vi "t162_ten_class_links.vi"() -> ()   [LabVIEW 2019]
doc: "Two classes, eight distinct methods and one vi.lib call: the method links carry contents 9 and 10 - a TAB and a line feed. Written as literal character references they stayed six characters long in the file, and LabVIEW refused the VI with Error 74 until 2026-10-12."
uses:
  Projects/LabVIEWMCP/experiments/aixml-without-grpc/tests/fixtures/Gauge/Gauge.lvclass
  Projects/LabVIEWMCP/experiments/aixml-without-grpc/tests/fixtures/Box/Box.lvclass
panel:
  out "trimmed":string
  out "width out":dbl
  out "offset out":dbl
  out "gain out":dbl
  out "name out":string
  in  "text":string
  in  "width":dbl
  in  "offset":dbl
  in  "gain":dbl
  in  "name":string
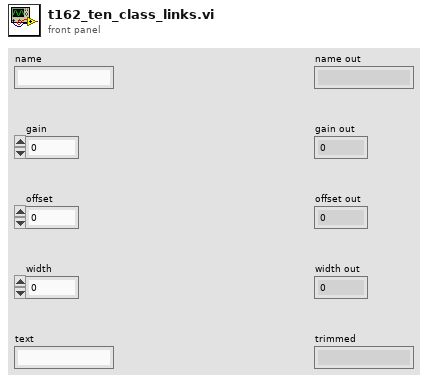
[diagram p1: front panel]
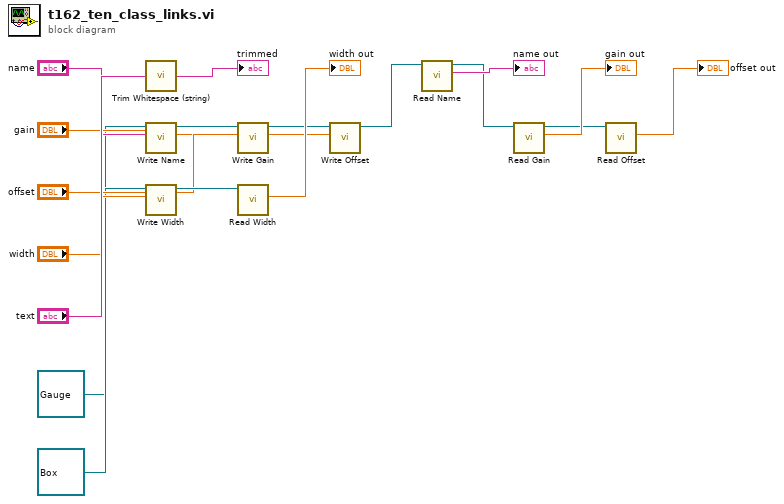
[diagram p0: block diagram]
diagram:
  n1 = call <vilib>:"Trim Whitespace (string).vi"("string"="text") -> ("trimmed string"=→"trimmed":string)  [unwired: 1 in]
  n2 = call-dynamic "Write Name.vi"("Name"="name", "Gauge in"=refnum<class "Gauge.lvclass"> refnum ("gauge")) -> ("Gauge out"=w9:refnum<class "Gauge.lvclass">)  [unwired: 8 in, 1 out]
  n3 = call-dynamic "Write Width.vi"("Width"="width", "Box in"=refnum<class "Box.lvclass"> refnum ("box")) -> ("Box out"=w17:refnum<class "Box.lvclass">)  [unwired: 8 in, 1 out]
  n4 = call-dynamic "Write Gain.vi"("Gain"="gain", "Gauge in"=w9) -> ("Gauge out"=w10:refnum<class "Gauge.lvclass">)  [unwired: 8 in, 1 out]
  n5 = call-dynamic "Read Width.vi"("Box in"=w17) -> ("Width"=→"width out":dbl)  [unwired: 8 in, 2 out]
  n6 = call-dynamic "Write Offset.vi"("Offset"="offset", "Gauge in"=w10) -> ("Gauge out"=w11:refnum<class "Gauge.lvclass">)  [unwired: 8 in, 1 out]
  n7 = call-dynamic "Read Name.vi"("Gauge in"=w11) -> ("Name"=→"name out":string, "Gauge out"=w12:refnum<class "Gauge.lvclass">)  [unwired: 8 in, 1 out]
  n8 = call-dynamic "Read Gain.vi"("Gauge in"=w12) -> ("Gain"=→"gain out":dbl, "Gauge out"=w14:refnum<class "Gauge.lvclass">)  [unwired: 8 in, 1 out]
  n9 = call-dynamic "Read Offset.vi"("Gauge in"=w14) -> ("Offset"=→"offset out":dbl)  [unwired: 8 in, 2 out]
